vi "Format Number Or NA.vi"(0 "Value":dbl, 5 "Format":string="%.;%.3f", 7 "NaN Text":string="n/a", 11 "error in":errorcluster) -> (4 "Text":string, 15 "error out":errorcluster)   [LabVIEW 2026]
doc: "Formats one number with a Format Into String format string, or returns NaN Text when the number is NaN, so a missing value never prints as garbage. Generic helper: knows nothing about the application. Pure function: error in is passed to error out unchanged."
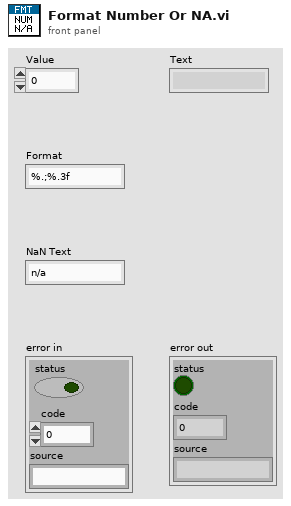
[diagram p1: front panel]
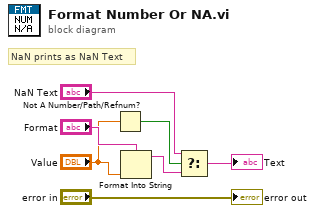
[diagram p0: block diagram]
diagram:
  # "NaN prints as NaN Text"
  n1 = Not A Number/Path/Refnum?(number/path/refnum="Value") -> (NaN/Path/Refnum?=w6:bool)
  n2 = Format Into String(format string="Format", "Value") -> (resulting string=w5:string)  [unwired: 2 in, 1 out]
  n3 = Select(t="NaN Text", s=w6, f=w5) -> (s? t:f=→"Text":string)
  "error out" <- "error in"
